vi "main.vi"() -> ()   [LabVIEW 2016]
panel:
  out "error out 2":errorcluster
  out "error out":errorcluster
  in  "vi path":path=path "D:/git/LabVIEW/ui-automation/labview-ui-testing/Prototype/ExeSubPanel/VI 2.vi"
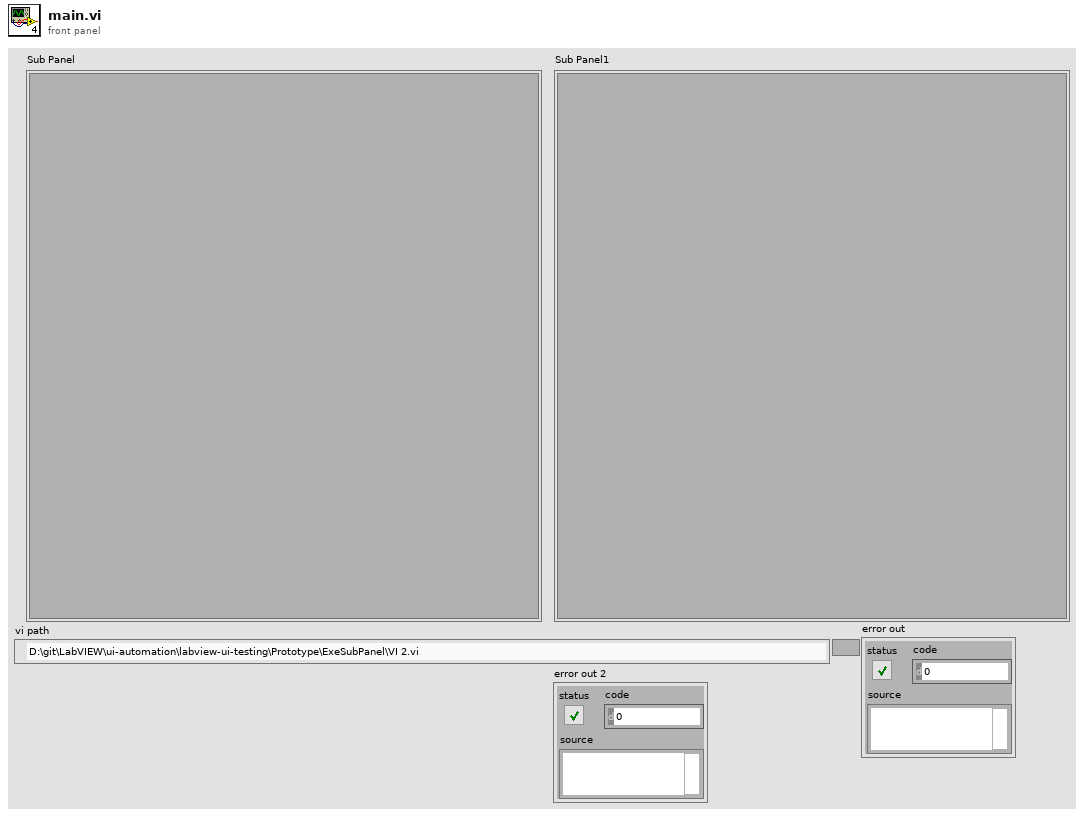
[diagram p1: front panel]
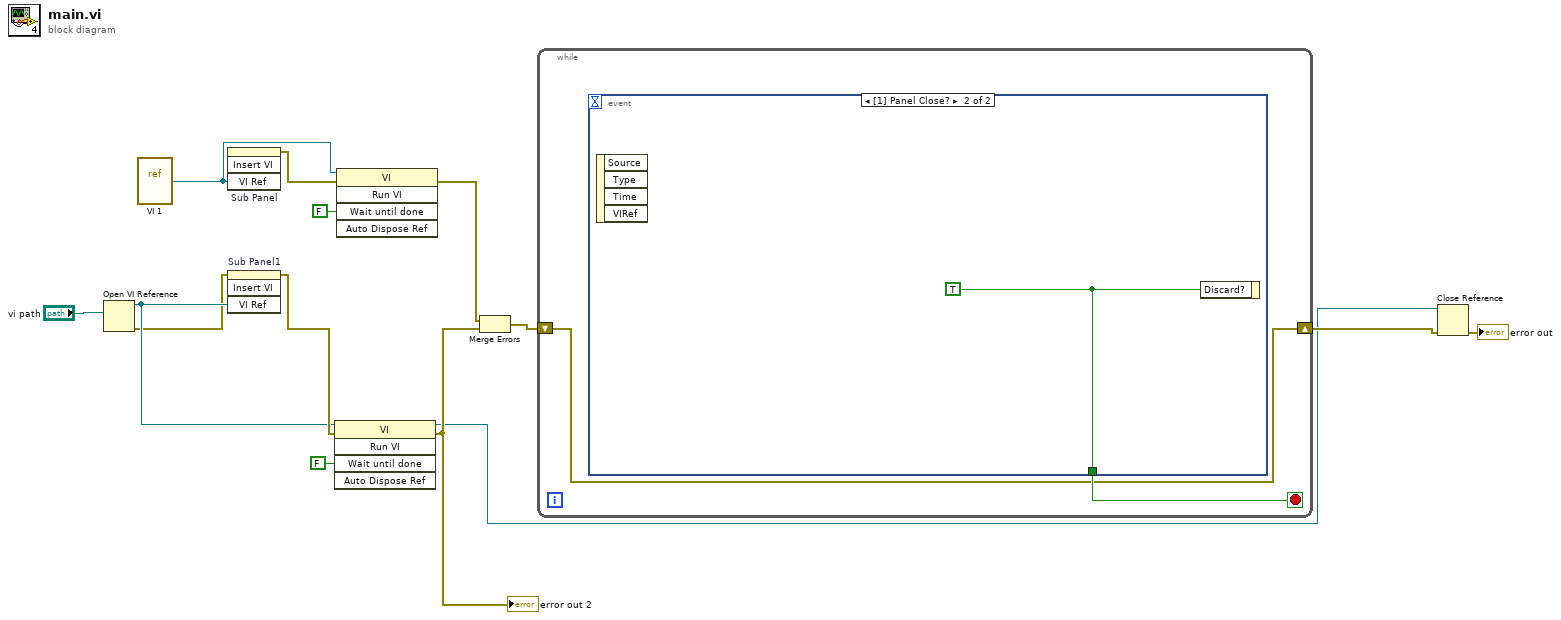
[diagram p0: block diagram]
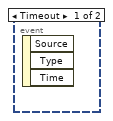
[diagram p2: hidden frame]
diagram:
  n1 = Open VI Reference(vi path="vi path") -> (vi reference=w7:refnum<vi>, error out=w6:errorcluster)  [unwired: 5 in]
  n2 = vi-ref "VI 1.vi"() -> (w14:refnum<vi>)
  n3 = invoke on="Sub Panel" class="SubPnl" method="Insert VI"("VI Ref"=w14) -> (error out=w13:errorcluster)  [unwired: 3 in, 3 out]
  n4 = invoke on="Sub Panel1" class="SubPnl" method="Insert VI"(error in=w6, "VI Ref"=w7) -> (error out=w10:errorcluster)  [unwired: 2 in, 3 out]
  n5 = invoke class="VI" method="Run VI"(reference=w7, error in=w10, "Wait until done"=FALSE ("Wait Until Done")) -> (reference out=w8:refnum<vi>, error out=w9:errorcluster)  [unwired: 2 in, 3 out]
  "error out 2" <- w9
  n6 = invoke class="VI" method="Run VI"(reference=w14, error in=w13, "Wait until done"=FALSE ("Wait Until Done")) -> (error out=w3:errorcluster)  [unwired: 2 in, 4 out]
  n7 = Merge Errors(w3, w9) -> (w4:errorcluster)
  n8 = while {
    shift-right: [w15] -> w11
    shift-left: w4 -> [w15]
    stop <- w16 stop-if-true
    n9 = event shown="[1] Panel Close?" {
      selector: _ -> [_ _]
      dyn-events: _ -> [_ _]
      timeout: _ -> [_ _]
      tunnel: [_ w17] -> w16
      event Timeout {
        n10 = event-data() -> ()  [unwired: 1 in, 3 out]
      }
      event Panel Close? {
        w17 = TRUE ("Discard?")
        n11 = event-data() -> ()  [unwired: 1 in, 4 out]
        n12 = event-data("Discard?"=w17) -> ()  [unwired: 1 in, 1 out]
      }
    }
  }
  n13 = Close Reference(reference=w8, error in (no error)=w11) -> (error out=→"error out":errorcluster)
